vi "RemoteVI Check Dirty Rects.vi"() -> (4 "labels":string[](array[string]), 6 "expected":string[](array[string]), 8 "actual":string[](array[string]), 10 "failures":i32)   [LabVIEW 2020]
doc: "Test support, generated by tests/caraya/build.py from tests/vectors/rects.json - do not edit. Calls RemoteVI Dirty Rects.vi once per vector: the vector's row-major pixels are reshaped to [height][width]; no previous capture is an empty previous array; rects are rendered x,y,w,h; in output order. Outputs, one element per vector: labels (the vector's name), expected (rendered from the vector), actual (the VI's result rendered the same way), and failures, the number of vectors whose expected and actual differ."
uses:
  source/RemoteVI.lvlib
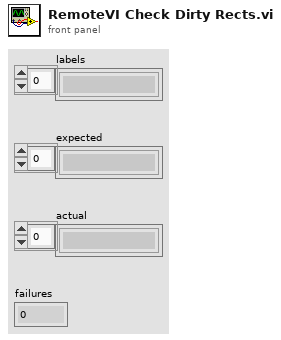
[diagram p1: front panel]
types:
  T1 = cluster{"name":string, "hasPrev":bool, "cur":u32[], "expect":string}[]
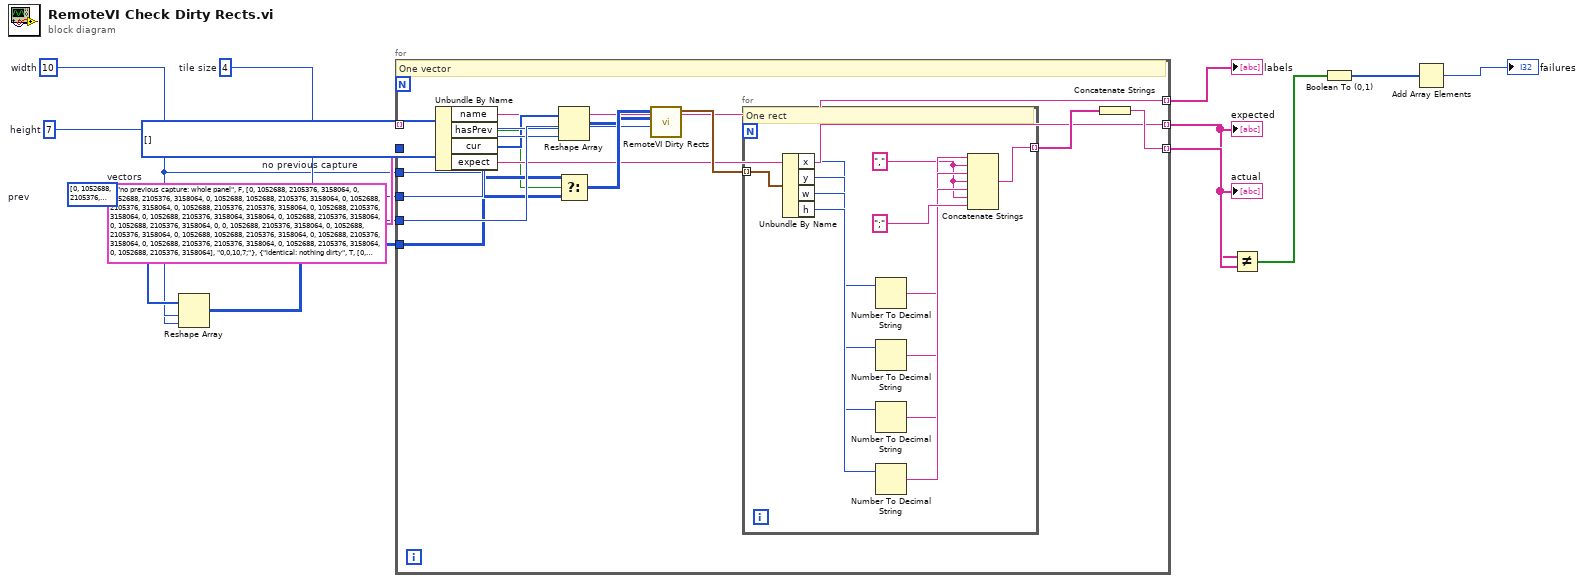
[diagram p0: block diagram]
diagram:
  w7 = T1 [{"name"="no previous capture: whole panel", "hasPrev"=FALSE, "cur"=[0, 1052688, 2105376, 3158064, 0, 1052688, 2105376, 3158064, 0, 1052688, 1052688, 2105376, 3158064, 0, 1052688, 2105376, 3158064, 0, 1052688, 2105376, 2105376, 3158064, 0, 1052688, 2105376, 3158064, 0, 1052688, 2105376, 3158064, 3158064, 0, 1052688, 2105376, 3158064, 0, 1052688, 2105376, 3158064, 0, 0, 1052688, 2105376, 3158064, 0, 1052688, 2105376, 3158064, 0, 1052688, 1052688, 2105376, 3158064, 0, 1052688, 2105376, 3158064, 0, 1052688, 2105376, 2105376, 3158064, 0, 1052688, 2105376, 3158064, 0, 1052688, 2105376, 3158064], "expect"="0,0,10,7;"}, {"name"="identical: nothing dirty", "hasPrev"=TRUE, "cur"=[0, 1052688, 2105376, 3158064, 0, 1052688, 2105376, 3158064, 0, 1052688, 1052688, 2105376, 3158064, 0, 1052688, 2105376, 3158064, 0, 1052688, 2105376, 2105376, 3158064, 0, 1052688, 2105376, 3158064, 0, 1052688, 2105376, 3158064, 3158064, 0, 1052688, 2105376, 3158064, 0, 1052688, 2105376, 3158064, 0, 0, 1052688, 2105376, 3158064, 0, 1052688, 2105376, 3158064, 0, 1052688, 1052688, 2105376, 3158064, 0, 1052688, 2105376, 3158064, 0, 1052688, 2105376, 2105376, 3158064, 0, 1052688, 2105376, 3158064, 0, 1052688, 2105376, 3158064], "expect"=""}, {"name"="one pixel in the first tile", "hasPrev"=TRUE, "cur"=[0, 1052688, 2105376, 3158064, 0, 1052688, 2105376, 3158064, 0, 1052688, 1052688, 14671839, 3158064, 0, 1052688, 2105376, 3158064, 0, 1052688, 2105376, 2105376, 3158064, 0, 1052688, 2105376, 3158064, 0, 1052688, 2105376, 3158064, 3158064, 0, 1052688, 2105376, 3158064, 0, 1052688, 2105376, 3158064, 0, 0, 1052688, 2105376, 3158064, 0, 1052688, 2105376, 3158064, 0, 1052688, 1052688, 2105376, 3158064, 0, 1052688, 2105376, 3158064, 0, 1052688, 2105376, 2105376, 3158064, 0, 1052688, 2105376, 3158064, 0, 1052688, 2105376, 3158064], "expect"="0,0,4,4;"}, {"name"="first and last tile of a row merge into one band", "hasPrev"=TRUE, "cur"=[16777215, 1052688, 2105376, 3158064, 0, 1052688, 2105376, 3158064, 0, 1052688, 1052688, 2105376, 3158064, 0, 1052688, 2105376, 3158064, 0, 1052688, 2105376, 2105376, 3158064, 0, 1052688, 2105376, 3158064, 0, 1052688, 2105376, 3158064, 3158064, 0, 1052688, 2105376, 3158064, 0, 1052688, 2105376, 3158064, 16777215, 0, 1052688, 2105376, 3158064, 0, 1052688, 2105376, 3158064, 0, 1052688, 1052688, 2105376, 3158064, 0, 1052688, 2105376, 3158064, 0, 1052688, 2105376, 2105376, 3158064, 0, 1052688, 2105376, 3158064, 0, 1052688, 2105376, 3158064], "expect"="0,0,10,4;"}, {"name"="clipped bottom-right tile", "hasPrev"=TRUE, "cur"=[0, 1052688, 2105376, 3158064, 0, 1052688, 2105376, 3158064, 0, 1052688, 1052688, 2105376, 3158064, 0, 1052688, 2105376, 3158064, 0, 1052688, 2105376, 2105376, 3158064, 0, 1052688, 2105376, 3158064, 0, 1052688, 2105376, 3158064, 3158064, 0, 1052688, 2105376, 3158064, 0, 1052688, 2105376, 3158064, 0, 0, 1052688, 2105376, 3158064, 0, 1052688, 2105376, 3158064, 0, 1052688, 1052688, 2105376, 3158064, 0, 1052688, 2105376, 3158064, 0, 1052688, 2105376, 2105376, 3158064, 0, 1052688, 2105376, 3158064, 0, 1052688, 2105376, 13619151], "expect"="8,4,2,3;"}, {"name"="one band per tile row", "hasPrev"=TRUE, "cur"=[0, 1052688, 2105376, 3158064, 0, 15724527, 2105376, 3158064, 0, 1052688, 1052688, 2105376, 3158064, 0, 1052688, 2105376, 3158064, 0, 1052688, 2105376, 2105376, 3158064, 0, 1052688, 2105376, 3158064, 0, 1052688, 2105376, 3158064, 3158064, 0, 1052688, 2105376, 3158064, 0, 1052688, 2105376, 3158064, 0, 0, 1052688, 2105376, 3158064, 0, 1052688, 2105376, 3158064, 0, 1052688, 1052688, 2105376, 3158064, 0, 1052688, 2105376, 3158064, 0, 1052688, 2105376, 14671839, 3158064, 0, 1052688, 2105376, 3158064, 0, 1052688, 2105376, 3158064], "expect"="4,0,4,4;0,4,4,3;"}]  # vectors
  w6 = u32[][] []  # no previous capture
  w4 = u32[] [0, 1052688, 2105376, 3158064, 0, 1052688, 2105376, 3158064, 0, 1052688, 1052688, 2105376, 3158064, 0, 1052688, 2105376, 3158064, 0, 1052688, 2105376, 2105376, 3158064, 0, 1052688, 2105376, 3158064, 0, 1052688, 2105376, 3158064, 3158064, 0, 1052688, 2105376, 3158064, 0, 1052688, 2105376, 3158064, 0, 0, 1052688, 2105376, 3158064, 0, 1052688, 2105376, 3158064, 0, 1052688, 1052688, 2105376, 3158064, 0, 1052688, 2105376, 3158064, 0, 1052688, 2105376, 2105376, 3158064, 0, 1052688, 2105376, 3158064, 0, 1052688, 2105376, 3158064]  # prev
  w3 = 4  # tile size
  w2 = 7  # height
  w1 = 10  # width
  n1 = Reshape Array(w4, w2, w1) -> (w5:u32[][])
  n2 = for {
    tunnel: w7 -> [w14] mode=indexing
    tunnel: w6 -> [w20]
    tunnel: w1 -> [w21]
    tunnel: w2 -> [w22]
    tunnel: w3 -> [w23]
    tunnel: w5 -> [w19]
    tunnel: [w15] -> w8 mode=indexing
    tunnel: [w18] -> w9 mode=indexing
    tunnel: [w28] -> w10 mode=indexing
    # "One vector"
    n3 = Unbundle By Name(w14) -> ("name"=w15:string, "hasPrev"=w16:bool, "cur"=w17:u32[], "expect"=w18:string)
    n4 = Reshape Array(w17, w22, w21) -> (w24:u32[][])
    n5 = Select(t=w19, s=w16, f=w20) -> (s? t:f=w25:u32[][])
    n6 = call "RemoteVI Dirty Rects.vi"("tile size"=w23, "current"=w24, "previous"=w25) -> ("rects"=w26:cluster{"x":i32, "y":i32, "w":i32, "h":i32}[])  [unwired: 8 in]
    n7 = for {
      tunnel: w26 -> [w29] mode=indexing
      tunnel: [w40] -> w27 mode=indexing
      w34 = ","
      # "One rect"
      n8 = Unbundle By Name(w29) -> ("x"=w30:i32, "y"=w31:i32, "w"=w32:i32, "h"=w33:i32)
      n9 = Number To Decimal String(number=w30) -> (decimal integer string=w35:string)  [unwired: 1 in]
      n10 = Number To Decimal String(number=w31) -> (decimal integer string=w36:string)  [unwired: 1 in]
      n11 = Number To Decimal String(number=w32) -> (decimal integer string=w37:string)  [unwired: 1 in]
      n12 = Number To Decimal String(number=w33) -> (decimal integer string=w38:string)  [unwired: 1 in]
      n13 = Concatenate Strings(w35, w34, w36, w34, w37, w34, w38, ";") -> (w40:string)
    }
    n14 = Concatenate Strings(w27) -> (w28:string)
  }
  "labels" <- w8
  "expected" <- w9
  "actual" <- w10
  n15 = Not Equal?(x=w9, y=w10) -> (x != y?=w11:bool[])
  n16 = Boolean To (0,1)(Boolean=w11) -> (0, 1=w12:i16[])
  n17 = Add Array Elements(numeric array=w12) -> (sum=→"failures":i16)
